vi "GetNotifyChangesEvent.vi"(8 "error in (no error)":errorcluster, 11 "ChangeNotifier in":refnum<class "ChangeNotifier.lvclass">) -> (0 "error out":errorcluster, 2 "notifyChangesEvent":refnum<user-event>, 3 "ChangeNotifier out":refnum<class "ChangeNotifier.lvclass">)   [LabVIEW 2024, in "ChangeNotifier.lvclass"]
uses:
  ChangeNotifier.lvclass
  ChangeNotifier.lvclass/ChangeNotifier.ctl
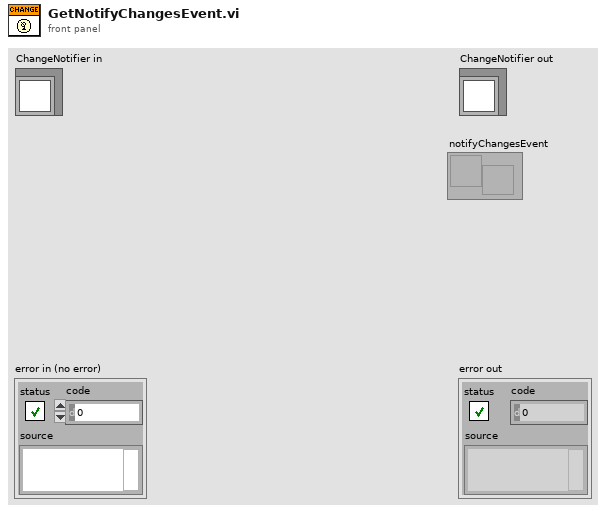
[diagram p1: front panel]
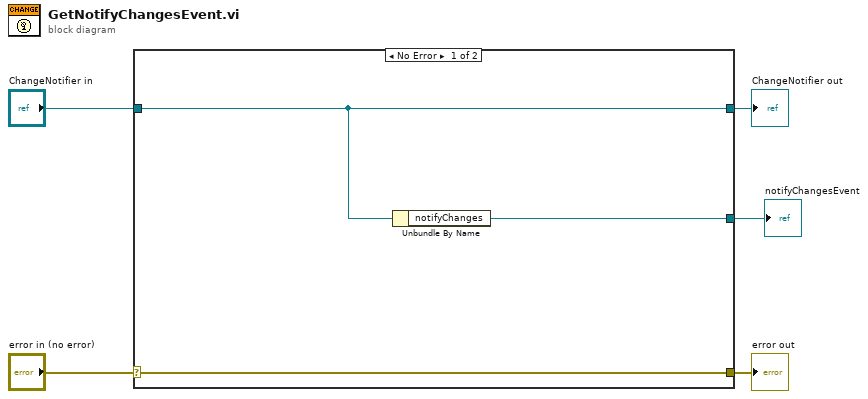
[diagram p0: block diagram]
diagram:
  n1 = case shown="No Error" "error in (no error)" {
    selector: "error in (no error)" -> [w8 w10]
    tunnel: [w8 w10] -> w4
    tunnel: [w7 w9] -> w2
    tunnel: "ChangeNotifier in" -> [w7 w9]
    tunnel: [w6 _] -> w1
    frame No Error {
      n2 = Unbundle By Name(w7) -> ("notifyChanges"=w6:refnum<user-event>)
    }
    frame Error {
    }
  }
  "error out" <- w4
  "ChangeNotifier out" <- w2
  "notifyChangesEvent" <- w1
